vi "Oscilloscope_myDAQ.vi"() -> ()   [LabVIEW 2026]
uses:
  <vilib>/DAQmx/read.llb/DAQmx Read (Analog 1D Wfm NChan NSamp).vi
  <vilib>/DAQmx/create/channels.llb/DAQmx Create Channel (AI-Voltage-Basic).vi
  <vilib>/DAQmx/configure/timing.llb/DAQmx Timing (Sample Clock).vi
  <vilib>/DAQmx/miscellaneous.llb/DAQmx Fill In Error Info.vi
  <vilib>/express/express analysis/Spectral/Block/exnSpectralBlock spectral measurements peak poly.vi
  <vilib>/express/express analysis/Spectral/Block/exnSpectralBlock spectral measurements peak DDT.vi
  <vilib>/measure/mamon.llb/Trigger Detection for 1 Channel.vi
  <vilib>/Waveform/WDTOps.llb/WDT Get Waveform Subset DBL.vi
  <vilib>/express/express analysis/Spectral/XNode/ExpressSpectralMeasurementsBlockNode.xnode
  <vilib>/measure/NI_MAPro.lvlib
panel:
  out "signal before  processing":waveform(dbl)[](graph)
  out "Samples I32":i32
  out "SINGLE CAPTURE":bool
  out "ARMED STATUS":bool
  in  "ARM/REARM":bool
  in  "Trigger Mode":enum16{"Auto", "Normal", "Single"}(ring)
  out "trigger location":dbl format="%#_2g"
  out "trigger detected":bool
  in  "trigger slope":u16(ring)=1 items=["Falling Edge", "Rising Edge"]
  in  "Trigger Source":enum16{"CH1", "CH2"}(ring)
  in  "Trigger Level (V)":dbl
  out "SPECTRUM CH2":dynamicdata(graph)
  out "SPECTRUM CH1":dynamicdata(graph)
  out "CH2 Period (ms)":dbl
  out "?":dbl
  out "Frequency 2":dbl
  out "Frequency":dbl
  out "RMS 2":dbl
  out "Positive Peak 2":dbl
  out "Peak to Peak 2":dbl
  out "Negative Peak 2":dbl
  out "Mean (DC) 2":dbl
  out "RMS":dbl
  out "Positive Peak":dbl
  out "Peak to Peak":dbl
  out "Negative Peak":dbl
  out "Mean (DC)":dbl
  in  "Time/Div (ms)":dbl=5.0 min=1.0 max=20.0 step=1.0
  in  "Volt/Div":dbl=0.5
  out "MAIN SCOPE":waveform(dbl)[](graph)
  in  "stop":bool
  # "CH2 MESURMENTS"
  # "CH1 MESURMENTS"
  # "Trigger settings"
  # "CH1 Period (ms)"
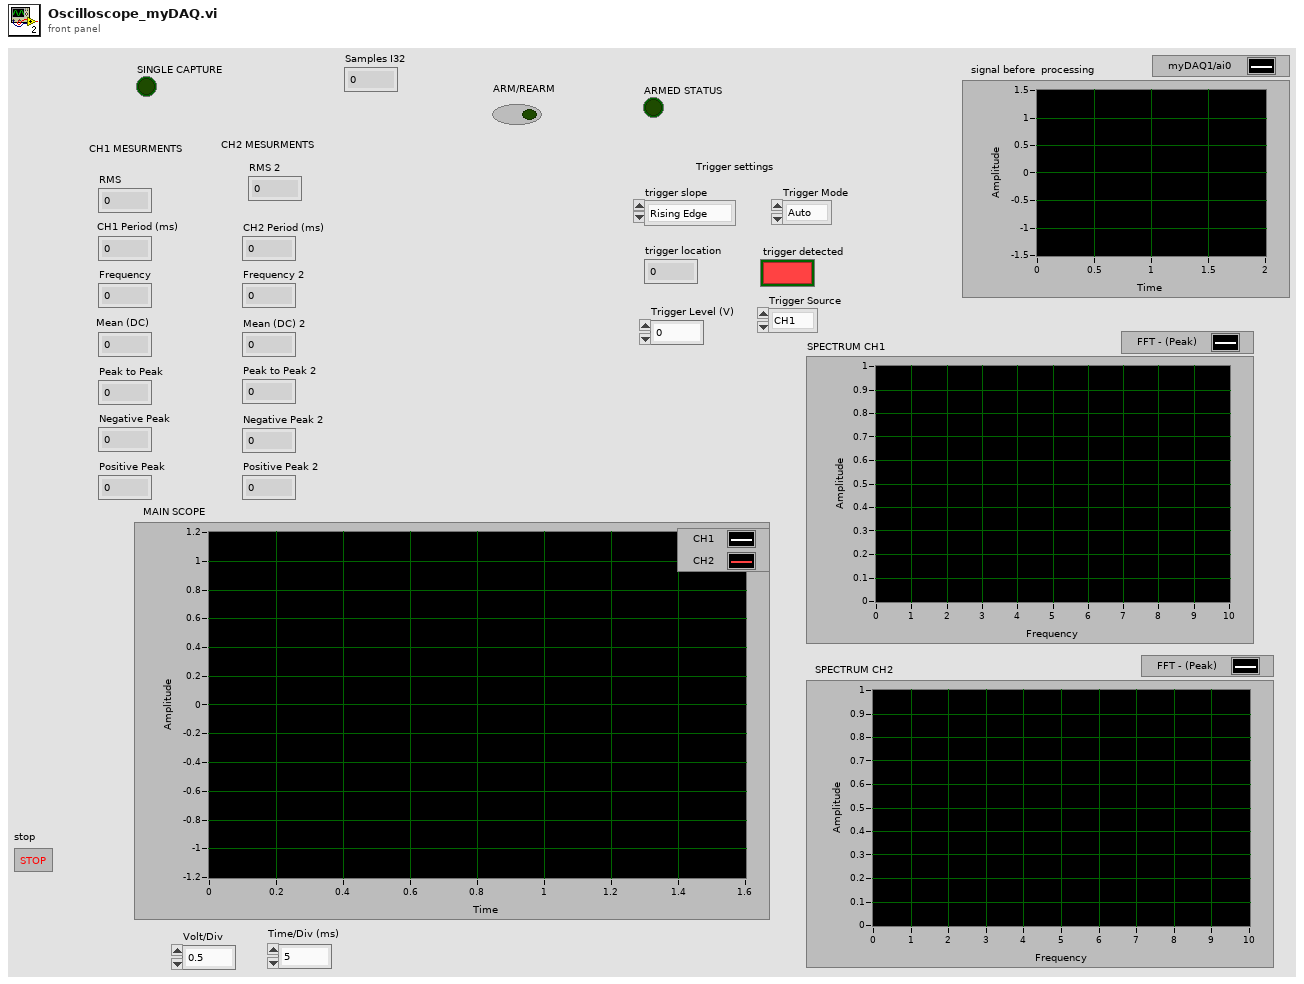
[diagram p1: front panel]
types:
  T1 = cluster{"averaging mode":u16, "weighting mode":u16, "number of averages":u32}
  T2 = cluster{"dB On (F)":bool, "unwrap phase (F)":bool, "convert to degree (F)":bool}
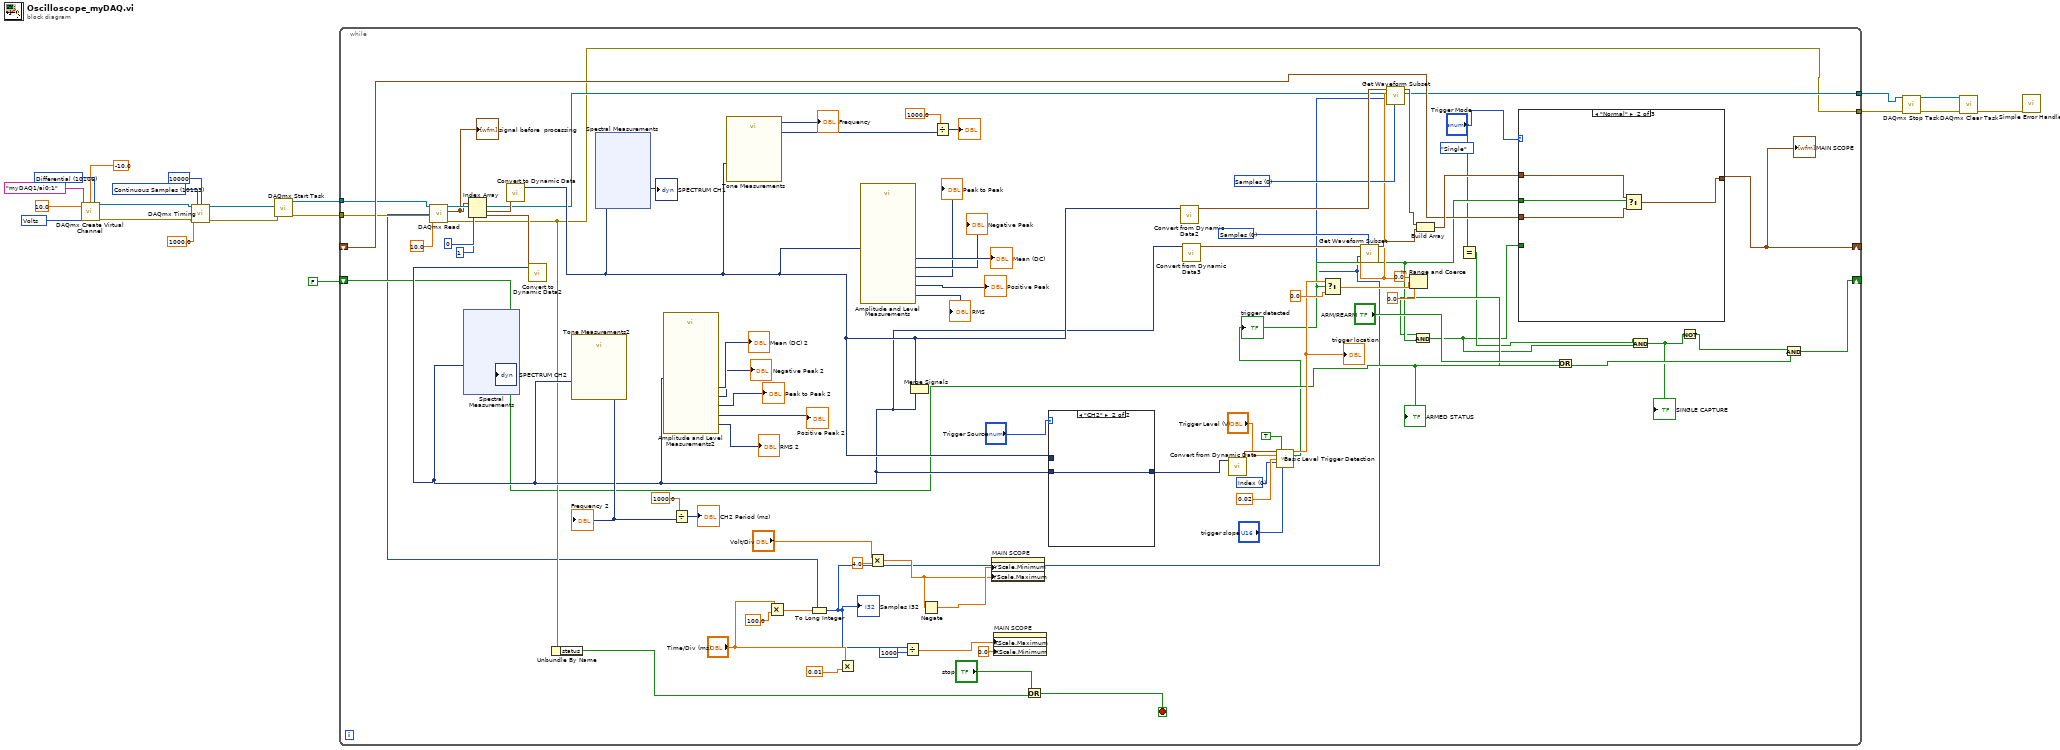
[diagram p0: block diagram]
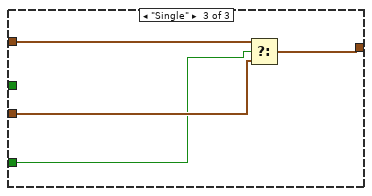
[diagram p3: hidden frame]
diagram:
  w13 = 10123 items=["Finite Samples"=10178, "Continuous Samples"=10123, "Hardware Timed Single Point"=12522] ("sample mode")
  w15 = 10348 items=["Volts"=10348, "From Custom Scale"=10065] ("units")
  w18 = 10106 items=["Default"=-1, "RSE"=10083, "NRSE"=10078, "Differential"=10106, "Pseudodifferential"=12529] ("input terminal configuration")
  n1 = call-poly <vilib>:"DAQmx Create Virtual Channel.vi"("maximum value"=10.0, "minimum value"=-10.0, "input terminal configuration"=w18, "physical channels"=tag "myDAQ1/ai0:1", "units"=w15) -> ("task out"=w19:refnum<k21>, "error out"=w10:errorcluster)  [unwired: 9 in]
  n2 = call-poly <vilib>:"DAQmx Timing.vi"("task/channels in"=w19, "sample mode"=w13, "samples per channel"=10000, "rate"=1000.0, "error in"=w10) -> ("task out"=w11:refnum<k21>, "error out"=w9:errorcluster)  [unwired: 9 in]
  n3 = call <vilib>:"DAQmx Start Task.vi"("task/channels in"=w11, "error in"=w9) -> ("task out"=w8:refnum<k21>, "error out"=w7:errorcluster)  [unwired: 12 in]
  n4 = while {
    shift-right: [w54] -> _
    shift-left: _ -> [w55]
    shift-right: [w36] -> _
    shift-left: FALSE -> [w38]
    tunnel: w8 -> [w53]
    tunnel: w7 -> [w52]
    tunnel: [w44] -> w6
    tunnel: [w43] -> w4
    stop <- w40 stop-if-true
    w65 = u16 0 items=["Samples", "Relative Time"] ("start/duration format")
    w66 = u16 0 items=["Samples", "Relative Time"] ("start/duration format")
    w71 = u16 0 items=["Index", "Time"] ("location mode")
    n5 = Multiply(x="Time/Div (ms)", y=100.0) -> (x*y=w26:dbl)
    n6 = To Long Integer(number=w26) -> (32bit integer=w24:i32)
    "Samples I32" <- w24
    n7 = call-poly <vilib>:"DAQmx Read.vi"("task/channels in"=w53, "number of samples per channel"=w24, "timeout"=10.0, "error in"=w52) -> ("task out"=w44:refnum<k21>, "data"=w25:waveform(dbl)[], "error out"=w43:errorcluster)  [unwired: 9 in]
    "signal before  processing" <- w25
    n8 = Index Array(array=w25, index #1=0 ("index"), index #2=1 ("index")) -> (element #1=w48:waveform(dbl), element #2=w47:waveform(dbl))
    n9 = call "Convert to Dynamic Data"("Waveform"=w48) -> ("Dynamic Data Type"=w46:dynamicdata)  [unwired: 3 in]
    n10 = call "Convert to Dynamic Data2"("Waveform"=w47) -> ("Dynamic Data Type"=w45:dynamicdata)  [unwired: 3 in]
    n11 = xnode "Spectral Measurements"("Signals"=w45) -> ("FFT - (Peak)"=→"SPECTRUM CH2":dynamicdata)  [unwired: 1 in, 2 out]
    n12 = Unbundle By Name(w43) -> ("status"=w41:bool)
    n13 = call "Tone Measurements2"("Signals"=w45) -> ("Frequency"=w81:dynamicdata)  [unwired: 9 in, 1 out]
    "Frequency 2" <- w81
    n14 = xnode "Spectral Measurements"("Signals"=w46) -> ("FFT - (Peak)"=→"SPECTRUM CH1":dynamicdata)  [unwired: 1 in, 2 out]
    n15 = call "Amplitude and Level Measurements2"("Signals"=w45) -> ("Mean (DC)"=→"Mean (DC) 2":dynamicdata, "RMS"=→"RMS 2":dynamicdata, "Negative Peak"=→"Negative Peak 2":dynamicdata, "Positive Peak"=→"Positive Peak 2":dynamicdata, "Peak to Peak"=→"Peak to Peak 2":dynamicdata)  [unwired: 9 in, 1 out]
    n16 = Divide(x=1000.0 ("y"), y=w81) -> (x/y=→"CH2 Period (ms)":dynamicdata)
    n17 = call "Tone Measurements"("Signals"=w46) -> ("Frequency"=w79:dynamicdata)  [unwired: 9 in, 1 out]
    "Frequency" <- w79
    n18 = Multiply(x="Time/Div (ms)", y=0.01) -> ()  [unwired: 1 out]
    n19 = call "Amplitude and Level Measurements"("Signals"=w46) -> ("Mean (DC)"=→"Mean (DC)":dynamicdata, "RMS"=→"RMS":dynamicdata, "Negative Peak"=→"Negative Peak":dynamicdata, "Positive Peak"=→"Positive Peak":dynamicdata, "Peak to Peak"=→"Peak to Peak":dynamicdata)  [unwired: 9 in, 1 out]
    n20 = Multiply(x="Volt/Div", y=4.0) -> (x*y=w96:dbl)
    n21 = Divide(x=w24, y=1000) -> (x/y=w22:dbl)
    n22 = Merge Signals(w46, w45) -> ()  [unwired: 1 out]
    n23 = Negate(x=w96) -> (-x=w97:dbl)
    n24 = Divide(x=1000.0 ("y"), y=w79) -> (x/y=→"?":dynamicdata)
    n25 = property on="MAIN SCOPE" class="WFGraph (strict)"("YScale.Minimum"=w97, "YScale.Maximum"=w96) -> ()  [unwired: 2 in, 2 out]
    n26 = property on="MAIN SCOPE" class="WFGraph (strict)"("XScale.Maximum"=w22, "XScale.Minimum"=0.0 ("X Scale.Range:Minimum")) -> ()  [unwired: 2 in, 2 out]
    n27 = Or(x="stop", y=w41) -> (x .or. y?=w40:bool)
    n28 = case shown="\"CH2\"" "Trigger Source" {
      tunnel: w46 -> [w109 _]
      tunnel: w45 -> [_ w110]
      tunnel: [w109 w110] -> w75
      frame "CH1", Default {
      }
      frame "CH2" {
      }
    }
    n29 = call "Convert from Dynamic Data2"("Dynamic Data Type"=w46) -> ("Waveform"=w68:waveform(dbl))  [unwired: 3 in]
    n30 = call "Convert from Dynamic Data3"("Dynamic Data Type"=w45) -> ("Waveform"=w67:waveform(dbl))  [unwired: 3 in]
    n31 = call "Convert from Dynamic Data"("Dynamic Data Type"=w75) -> ("Waveform"=w74:waveform(dbl))  [unwired: 3 in]
    n32 = call-poly <vilib>:"Basic Level Trigger Detection.vi"("signal in"=w74, "reset"=TRUE, "level"="Trigger Level (V)", "hysteresis"=0.02, "location mode"=w71, "trigger slope"="trigger slope") -> ("trigger location"=w61:dbl, "trigger detected?"=w35:bool)  [unwired: 7 in, 1 out]
    "trigger detected" <- w35
    "trigger location" <- w61
    n33 = Select(t=w61, s=w35, f=0.0) -> (s? t:f=w60:dbl)
    n34 = In Range and Coerce(upper limit=0.0, x=w60, lower limit=0.0) -> (coerced(x)=w57:dbl)  [unwired: 1 out]
    n35 = call-poly <vilib>:"Get Waveform Subset.vi"("start/duration format"=w65, "duration"=w24, "start samples/time"=w57, "waveform in"=w67) -> ("waveform out"=w63:waveform(dbl))  [unwired: 2 in, 3 out]
    n36 = call-poly <vilib>:"Get Waveform Subset.vi"("start/duration format"=w66, "duration"=w24, "start samples/time"=w57, "waveform in"=w68) -> ("waveform out"=w64:waveform(dbl))  [unwired: 2 in, 3 out]
    n37 = Build Array(w64, w63) -> (w56:waveform(dbl)[])
    n38 = Equal?(x="Trigger Mode", y=enum16{"Auto", "Normal", "Single"}."Single") -> (x = y?=w31:bool)
    n39 = Or(x="ARM/REARM", y=w38) -> (x .or. y?=w34:bool)
    n40 = And(x=w34, y=w35) -> (x .and. y?=w29:bool)
    n41 = case shown="\"Normal\"" "Trigger Mode" {
      tunnel: [w100 w102 w105] -> w54
      tunnel: w56 -> [w100 w104 w108]
      tunnel: w55 -> [_ w103 w107]
      tunnel: w29 -> [_ _ w106]
      tunnel: w35 -> [_ w101 _]
      frame "Auto", Default {
      }
      frame "Normal" {
        n42 = Select(t=w104, s=w101, f=w103) -> (s? t:f=w102:waveform(dbl)[])
      }
      frame "Single" {
        n43 = Select(t=w108, s=w106, f=w107) -> (s? t:f=w105:waveform(dbl)[])
      }
    }
    "MAIN SCOPE" <- w54
    n44 = And(x=w31, y=w29) -> (x .and. y?=w30:bool)
    "SINGLE CAPTURE" <- w30
    n45 = Not(x=w30) -> (.not. x?=w37:bool)
    n46 = And(x=w37, y=w34) -> (x .and. y?=w36:bool)
    "ARMED STATUS" <- w38
  }
  n47 = call <vilib>:"DAQmx Stop Task.vi"("task/channels in"=w6, "error in"=w4) -> ("task out"=w5:refnum<k21>, "error out"=w3:errorcluster)  [unwired: 12 in]
  n48 = call <vilib>:"DAQmx Clear Task.vi"("task in"=w5, "error in"=w3) -> ("error out"=w2:errorcluster)  [unwired: 13 in]
  n49 = call <vilib>:"Simple Error Handler.vi"("error in (no error)"=w2) -> ()  [unwired: 4 in, 5 out]
